vi "Verdict.vi"(11 "Tension":dbl) -> (3 "OK":bool)   [LabVIEW 2026]
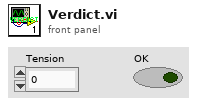
[diagram p1: front panel]
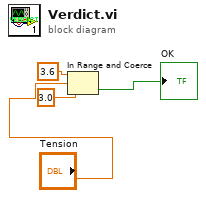
[diagram p0: block diagram]
diagram:
  n1 = In Range and Coerce(upper limit=3.6, x="Tension", lower limit=3.0) -> (In Range?=→"OK":bool)  [unwired: 1 out]
